vi "Check Labels.vi"(0 "Histogram in":refnum<class "Histogram.lvclass">, 11 "error in (no error)":errorcluster, 12 "Labels":map{string, string}(c390)) -> (4 "Samples":map{string, refnum<class "Sample.lvclass">}(c390), 6 "Valid Labels":bool, 8 "Label Values":string[](array[string]), 15 "error out":errorcluster)   [LabVIEW 2020, in "Metrics.lvlib" / "Histogram.lvclass"]
uses:
  Histogram.lvclass
  C:/Github-locals/PromVIEW/src/metrics/metric/Metric.lvclass
  sample/Sample.lvclass
  metric/Metric.lvclass/Metric.ctl
  metric/Read Samples.vi
  metric/Read Label Names.vi
  Histogram.lvclass/Histogram.ctl
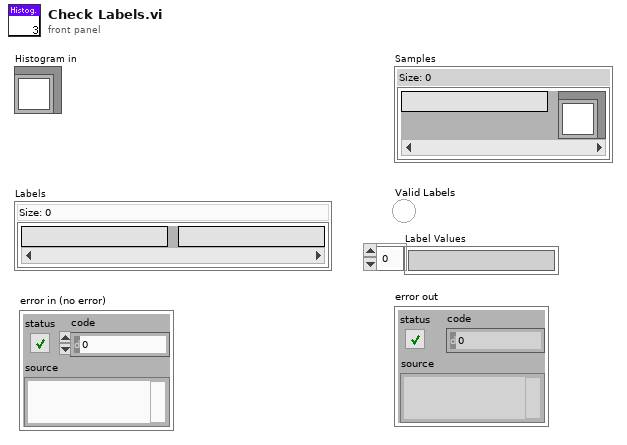
[diagram p1: front panel]
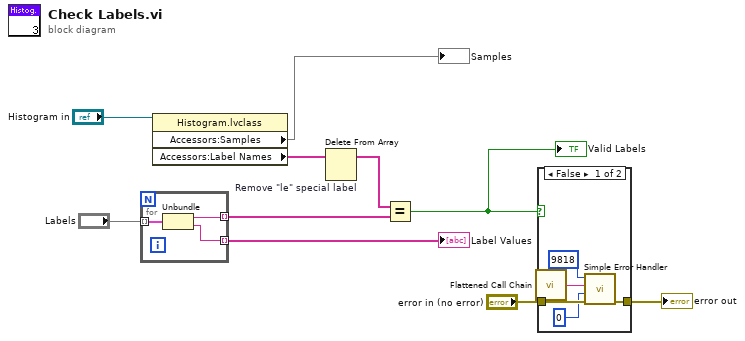
[diagram p0: block diagram]
diagram:
  n1 = for {
    tunnel: [w13] -> w9 mode=indexing
    tunnel: [w12] -> w6 mode=indexing
    tunnel: "Labels" -> [w11] mode=indexing
    n2 = Unbundle(w11) -> ("labelname"=w13:string, "labelvalue"=w12:string)
  }
  "Label Values" <- w6
  n3 = property class="Histogram.lvclass"(reference="Histogram in") -> ("Accessors:Samples"=→"Samples":map{string, refnum<class "Sample.lvclass">}, "Accessors:Label Names"=w5:string[])  [unwired: 1 in, 2 out]
  n4 = Delete From Array "Remove \"le\" special label"(array=w5) -> (array with subset deleted=w7:string[])  [unwired: 2 in, 1 out]
  n5 = Equal?(x=w7, y=w9) -> (x = y?=w1:bool)
  "Valid Labels" <- w1
  n6 = case shown="False" w1 {
    tunnel: "error in (no error)" -> [w18 w19]
    tunnel: [w14 w19] -> w2
    frame False {
      n7 = call "Flattened Call Chain.vi"() -> ("Flattened Call Chain"=w16:string)  [unwired: 5 in]
      n8 = call <vilib>:"Simple Error Handler.vi"("error code (no error:0)"=9818, "error source (\" \")"=w16, "type of dialog (OK msg:1)"=0 ("error code (no error:0)"), "error in (no error)"=w18) -> ("error out"=w14:errorcluster)  [unwired: 1 in, 4 out]
    }
    frame True {
    }
  }
  "error out" <- w2
